vi "Calculate Output Sampling.vi"(10 "sampling info":cluster{"Fs":dbl, "#s":dbl}={"Fs"=204800.0, "#s"=20480.0}, 11 "Cfg_REF":T2 {"Roll-Off" min=1 max=4; "TC" min=1e-06 max=100.0 format="%#_3p"; "Phase" format="%#_3g"; "Frequency" min=1e-06 max=102400.0 format="%#_6p"; "Channel" min=1}) -> (2 "Filter Parameters":T1, 3 "Cfg_REF out":T2 {"Roll-Off" min=1 max=4; "TC" min=1e-06 max=100.0 format="%#_3p"; "Phase" format="%#_3g"; "Frequency" min=1e-06 max=102400.0 format="%#_6p"; "Channel" min=1})   [LabVIEW 2019, in "Instrument.Lockin.lvlib" / "Instrument.Lockin.lvclass"]
uses:
  Instrument.Lockin.lvclass
  Instrument.DAQ/Typedefs/REF.Channel--Cluster--Array.ctl
  Instrument.DAQ/Typedefs/REF.Channel--Cluster.ctl
  DSP/DSP.lvclass
  Instrument.DAQ/Instrument.DAQ.lvclass
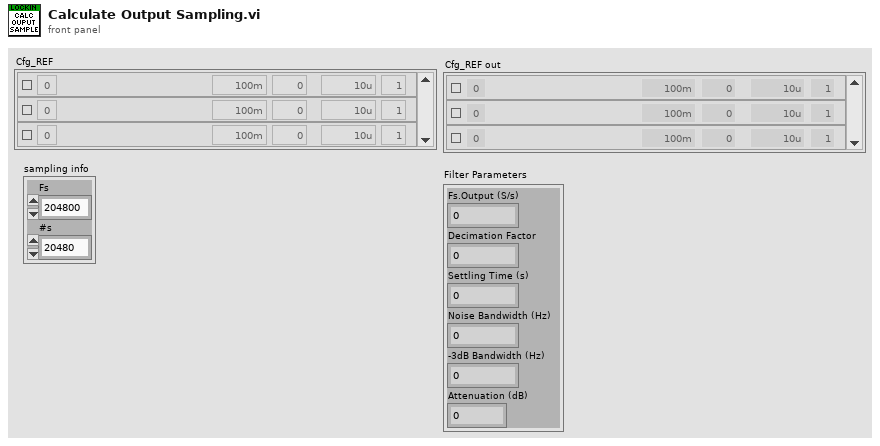
[diagram p1: front panel]
types:
  T1 = cluster{"Fs.Output (S/s)":dbl, "Decimation Factor":i32, "Settling Time (s)":dbl, "Noise Bandwidth (Hz)":dbl, "-3dB Bandwidth (Hz)":dbl, "Attenuation (dB)":dbl}
  T2 = typedef "Instrument.Lockin.lvlib/Instrument.DAQ.lvclass/REF.Channel--Cluster--Array.ctl" = T3[]
  T3 = typedef "Instrument.Lockin.lvlib/Instrument.DAQ.lvclass/REF.Channel--Cluster.ctl" = cluster{"Enable?":bool, "Channel":i32, "Frequency":dbl, "Phase":dbl, "TC":dbl, "Roll-Off":i32}
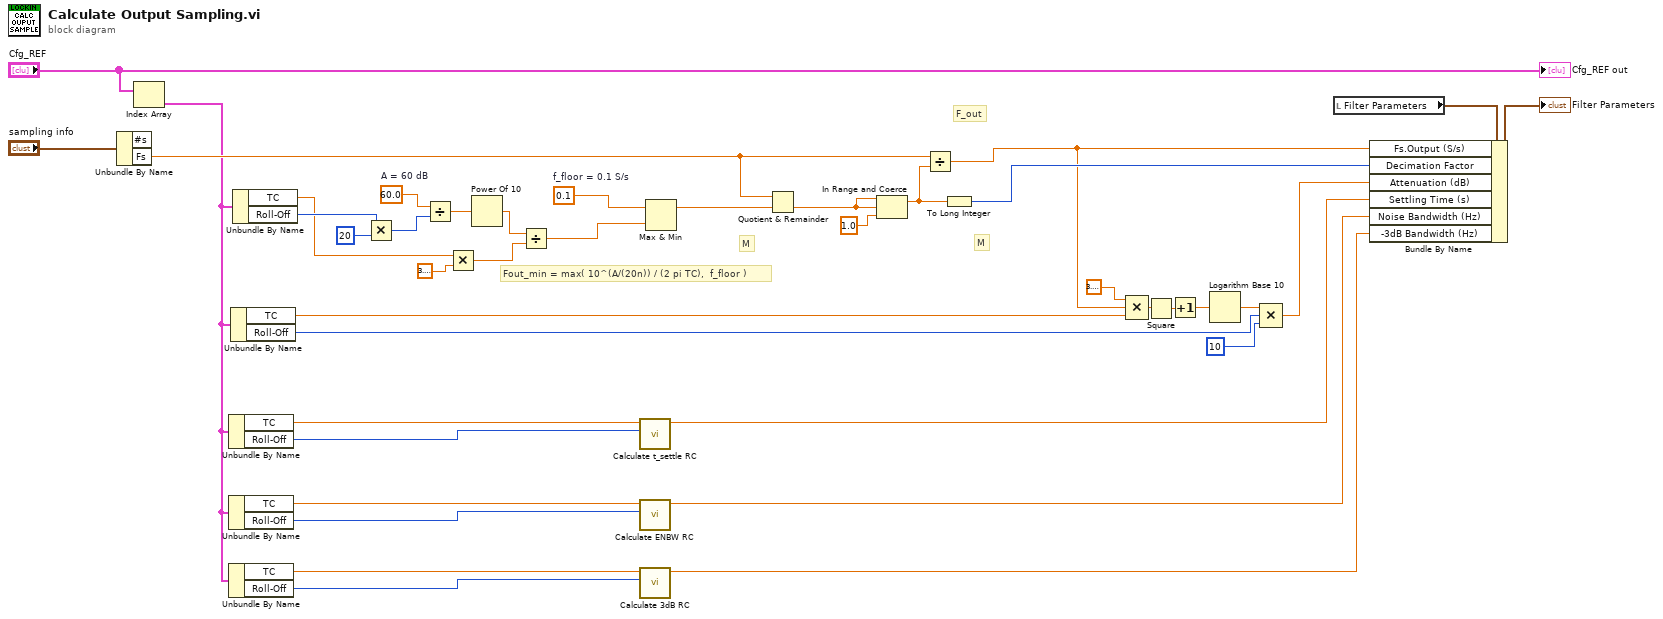
[diagram p0: block diagram]
diagram:
  w21 = 60.0  # A = 60 dB
  w26 = 0.1  # f_floor = 0.1 S/s
  # "M"
  # "F_out"
  # "Fout_min = max( 10^(A/(20n)) / (2 pi TC),  f_floor )"
  # "M"
  n1 = Unbundle By Name("sampling info") -> ("Fs"=w35:dbl)  [unwired: 1 out]
  n2 = Index Array(array="Cfg_REF") -> (element=w33:T3)  [unwired: 1 in]
  n3 = Unbundle By Name(w33) -> ("TC"=w28:dbl, "Roll-Off"=w27:i32)
  n4 = Unbundle By Name(w33) -> ("TC"=w30:dbl, "Roll-Off"=w29:i32)
  n5 = Unbundle By Name(w33) -> ("TC"=w32:dbl, "Roll-Off"=w31:i32)
  n6 = Unbundle By Name(w33) -> ("TC"=w13:dbl, "Roll-Off"=w8:i32)
  n7 = Unbundle By Name(w33) -> ("TC"=w20:dbl, "Roll-Off"=w25:i32)
  n8 = Multiply(x=w25, y=20) -> (x*y=w22:i32)
  n9 = Divide(x=w21, y=w22) -> (x/y=w23:dbl)
  n10 = Multiply(x=w20, y=3.141592653589793) -> (x*y=w17:dbl)
  n11 = Power Of 10(x=w23) -> (10^x=w18:dbl)
  n12 = Divide(x=w18, y=w17) -> (x/y=w16:dbl)
  n13 = call "Calculate t_settle RC.vi"("filter order"=w27, "time constant (s)"=w28) -> ("f -3 dB (Hz)"=w37:dbl)  [unwired: 9 in]
  n14 = call "Calculate ENBW RC.vi"("filter order"=w29, "time constant (s)"=w30) -> ("ENBW (Hz)"=w38:dbl)  [unwired: 9 in]
  n15 = call "Calculate 3dB RC.vi"("filter order"=w31, "time constant (s)"=w32) -> ("f -3 dB (Hz)"=w39:dbl)  [unwired: 9 in]
  n16 = Max & Min(x=w26, y=w16) -> (max(x,y)=w15:dbl)  [unwired: 1 out]
  n17 = Quotient & Remainder(x=w35, y=w15) -> (floor(x/y)=w4:dbl)  [unwired: 1 out]
  n18 = In Range and Coerce(upper limit=w4, x=w4, lower limit=1.0) -> (coerced(x)=w3:dbl)  [unwired: 1 out]
  n19 = Divide(x=w35, y=w3) -> (x/y=w1:dbl)
  n20 = To Long Integer(number=w3) -> (32bit integer=w2:i32)
  n21 = Compound Arithmetic op=MULTIPLY(3.141592653589793, w1, w13) -> (w11:dbl)
  n22 = Square(x=w11) -> (x^2=w5:dbl)
  n23 = Increment(x=w5) -> (x+1=w10:dbl)
  n24 = Logarithm Base 10(1:w10) -> (0:w9:dbl)
  n25 = Compound Arithmetic op=MULTIPLY(w9, w8, 10 ("y")) -> (w36:dbl)
  n26 = local read "Filter Parameters"() -> (w41:T1)
  n27 = Bundle By Name(cluster=w41, "Fs.Output (S/s)"=w1, "Decimation Factor"=w2, "Attenuation (dB)"=w36, "Settling Time (s)"=w37, "Noise Bandwidth (Hz)"=w38, "-3dB Bandwidth (Hz)"=w39) -> (→"Filter Parameters":T1)
  "Cfg_REF out" <- "Cfg_REF"
